vi "COS.vi"(3 "加速度":dbl format="%#_13g", 4 "間隔":i32, 5 "距離":i32) -> (1 "加速度曲線":dbl[](array[numeric]), 2 "週期曲線":u32[](array[numeric]))   [LabVIEW 2019]
panel:
  out "output array":dbl[](array[numeric])
  out "x-y":i32
  out "Waveform Graph":u32[](graph)
  out "Waveform Chart":u32[](graph)
  out "x+1":i32
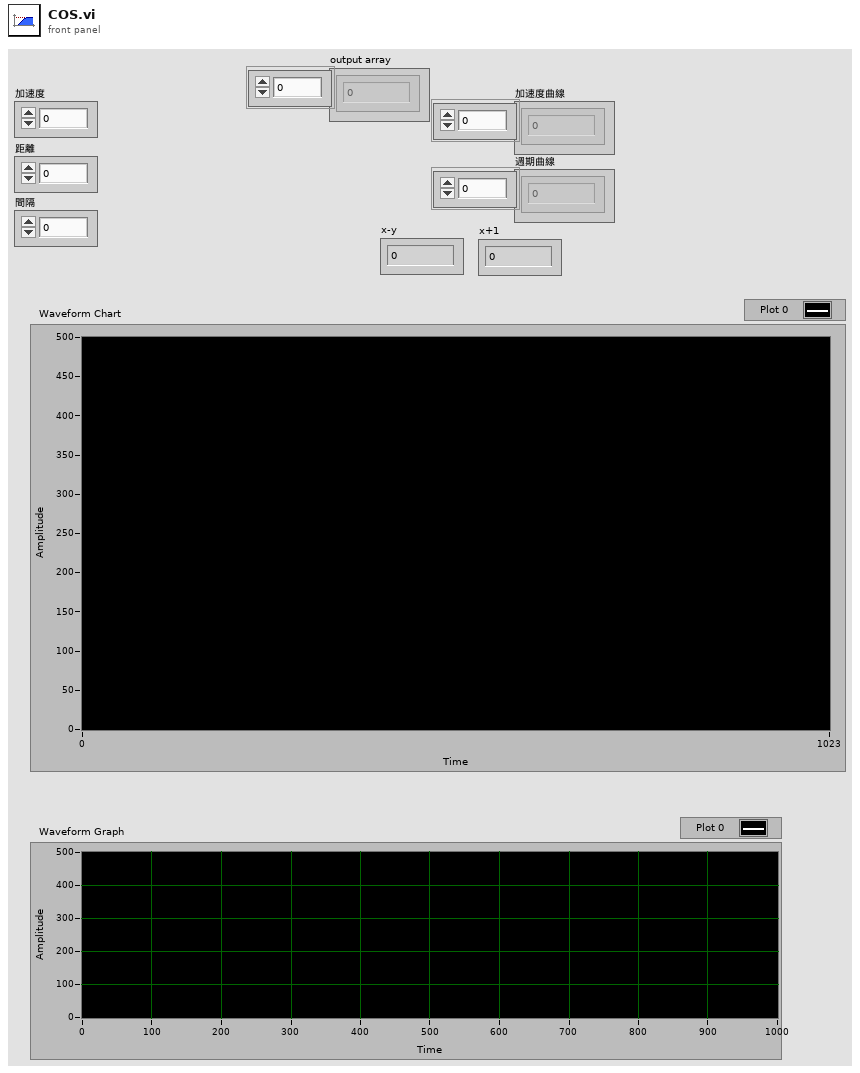
[diagram p1: front panel]
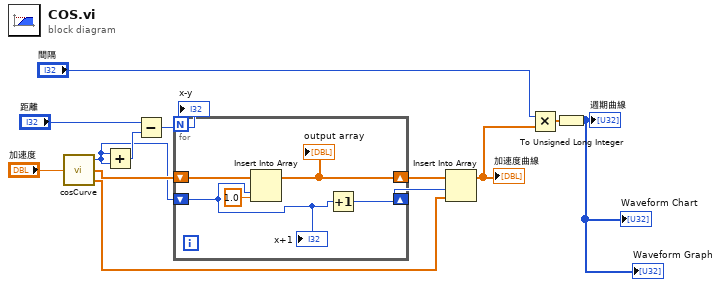
[diagram p0: block diagram]
diagram:
  n1 = call "cosCurve.vi"("x"="加速度") -> ("減速cos曲線"=w6:dbl[], "加速cos曲線"=w9:dbl[], "曲線迴圈數"=w8:i32)  [unwired: 2 in]
  n2 = Add(x=w8, y=w8) -> (x+y=w11:i32)
  n3 = Subtract(x="距離", y=w11) -> (x-y=w10:i32)
  "x-y" <- w10
  n4 = for {
    N: w10 -> [_]
    shift-right: [w14] -> w5
    shift-left: w8 -> [w15]
    shift-right: [w16] -> w7
    shift-left: w9 -> [w18]
    n5 = Insert Into Array(array=w18, index=w15, new element=1.0 ("new element/subarray")) -> (w16:dbl[])
    "output array" <- w16
    n6 = Increment(x=w15) -> (x+1=w14:i32)
    "x+1" <- w15
  }
  n7 = Insert Into Array(array=w7, index=w5, new element=w6) -> (w4:dbl[])
  "加速度曲線" <- w4
  n8 = Multiply(x="間隔", y=w4) -> (x*y=w2:dbl[])
  n9 = To Unsigned Long Integer(number=w2) -> (unsigned 32bit integer=→"週期曲線" →"Waveform Chart" →"Waveform Graph":u32[])
